vi "Report - PWP Stabilization Report.vi"(8 "error in":errorcluster, 11 "Fileid":string) -> (0 "error out":errorcluster)   [LabVIEW 2019]
uses:
  Controls/Report - State.ctl
  Controls/Report - Data Structure.ctl
  <vilib>/httpClient/ClientHandle.ctl
  Controls/FGV States.ctl
  Controls/eFGV States.ctl
  Controls/JSON - Fileid.ctl
  Controls/JSON - Report.ctl
  <vilib>/Utility/sysdir.llb/System Directory Type.ctl
  <vilib>/httpClient/POSTBuffer.vi
  <userlib>/_OpenG.lib/array/array.llb/Remove Duplicates from 1D Array (String)__ogtk.vi
  <userlib>/_OpenG.lib/array/array.llb/Delete Elements from 1D Array (String)__ogtk.vi
  <vilib>/Utility/config.llb/Read Key (String).vi
  <vilib>/httpClient/LabVIEWHTTPClient.lvlib
  <vilib>/Utility/config.llb/NI_LVConfig.lvlib
panel:
  in  "Plot":bool
  out "Current stage":T1
  in  "Back":bool
  in  "Forward":bool
  in  "Pages":u32
  out "Total":u32
  out "data":T2(array[cluster])
  in  "Cancel":bool
  in  "Generate":bool
  in  "Search":string
  in  "Listbox":i32(listbox)=-1 caption="Select File to Export"
  # "of"
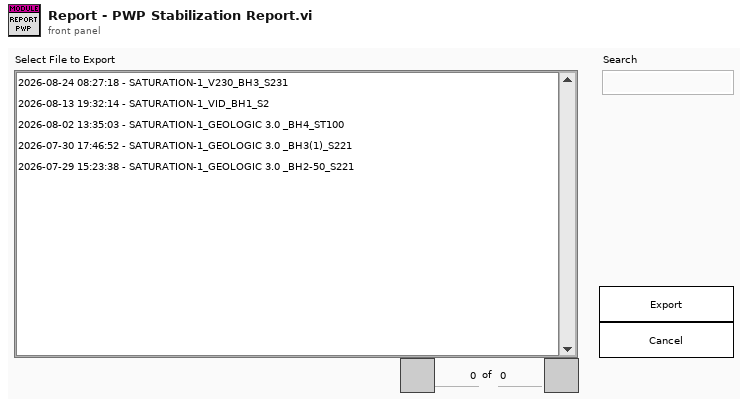
[diagram p1: front panel]
types:
  T1 = typedef "Report - State.ctl" = enum16{"Init", "Get File List", "Get Station Name", "Parse File List", "Idle", "Prepare to Generate", "Get Report", "Parse Report", "Get Data", "View T90", "Parse Data", "Convert to Excel", "Clean Up", "Close"}
  T2 = cluster{"id":string, "created_date":string, "testname":string, "jobno":string, "jobdesc":string, "sampleid":string, "date":string, "specimentno":string, "depth":string, "height":string, "diameter":string, "weight":string, "done":string}[]
  T3 = typedef "eFGV States.ctl" = enum16{"Init", "Read", "Write", "Exit"}
  T4 = typedef "FGV States.ctl" = enum16{"Read", "Write"}
  T5 = typedef "Report - Data Structure.ctl" = cluster{"API Ref":T6, "FileList":string[][], "Fileid":string, "testname":string[], "testtype":string[], "tdms":refnum<k34>, "TDMS Path":path, "tdms_path":string, "excel_path":string, "Excel Path":path, "List Name":string[], "Station Name":string[], "Plot":bool, "Tangent Point":string}
  T6 = typedef "LabVIEWHTTPClient.lvlib/ClientHandle.ctl" = refnum<k1>
  T7 = enum32{"Invalid", "Default", "Floating", "Floating/Auto-Hide", "Modal"}
  T8 = enum32{"Invalid", "Standard", "Closed", "Hidden", "Minimized", "Maximized"}
  T9 = typedef "JSON - Fileid.ctl" = cluster{"status":string, "data":cluster{"id":string, "created_date":string, "testname":string, "jobno":string, "jobdesc":string, "sampleid":string, "date":string, "specimentno":string, "depth":string, "height":string, "diameter":string, "weight":string, "done":string}[]}
  T10 = typedef "JSON - Report.ctl" = cluster{"status":string, "data":cluster{"testname":string, "testtype":string, "stage":string}[]}
  T11 = enum16{"open", "open or create", "create or replace", "create", "open (read-only)"}
  T12 = typedef "eventvkey.ctl" = enum16{"ASCII", "Enter", "Return", "Shift", "Ctrl", "Alt", "Cmd", "Opt", "Caps", "NumLock", "Clear", "Break", "Up", "Down", "Left", "Right", "Insert", "Delete", "Home", "End", "PageUp", "PageDown", "Escape", "Help", "Pause", "ScrollLock", "F1", "F2", "F3", "F4", "F5", "F6", "F7", "F8", "F9", "F10", "F11", "F12", "F13", "F14", "F15", "F16", "F17", "F18", "F19", "F20", "F21", "F22", "F23", "F24", "Play", "VolumeUp", "VolumeDown", "Mute", "Two Byte Char"}
  T13 = cluster{"testname":string, "testtype":string, "stage":string}[]
  T14 = typedef "System Directory Type.ctl" = i32
  T15 = typedef "NI_LVConfig.lvlib/Config Data RefNum.ctl" = refnum<k1>
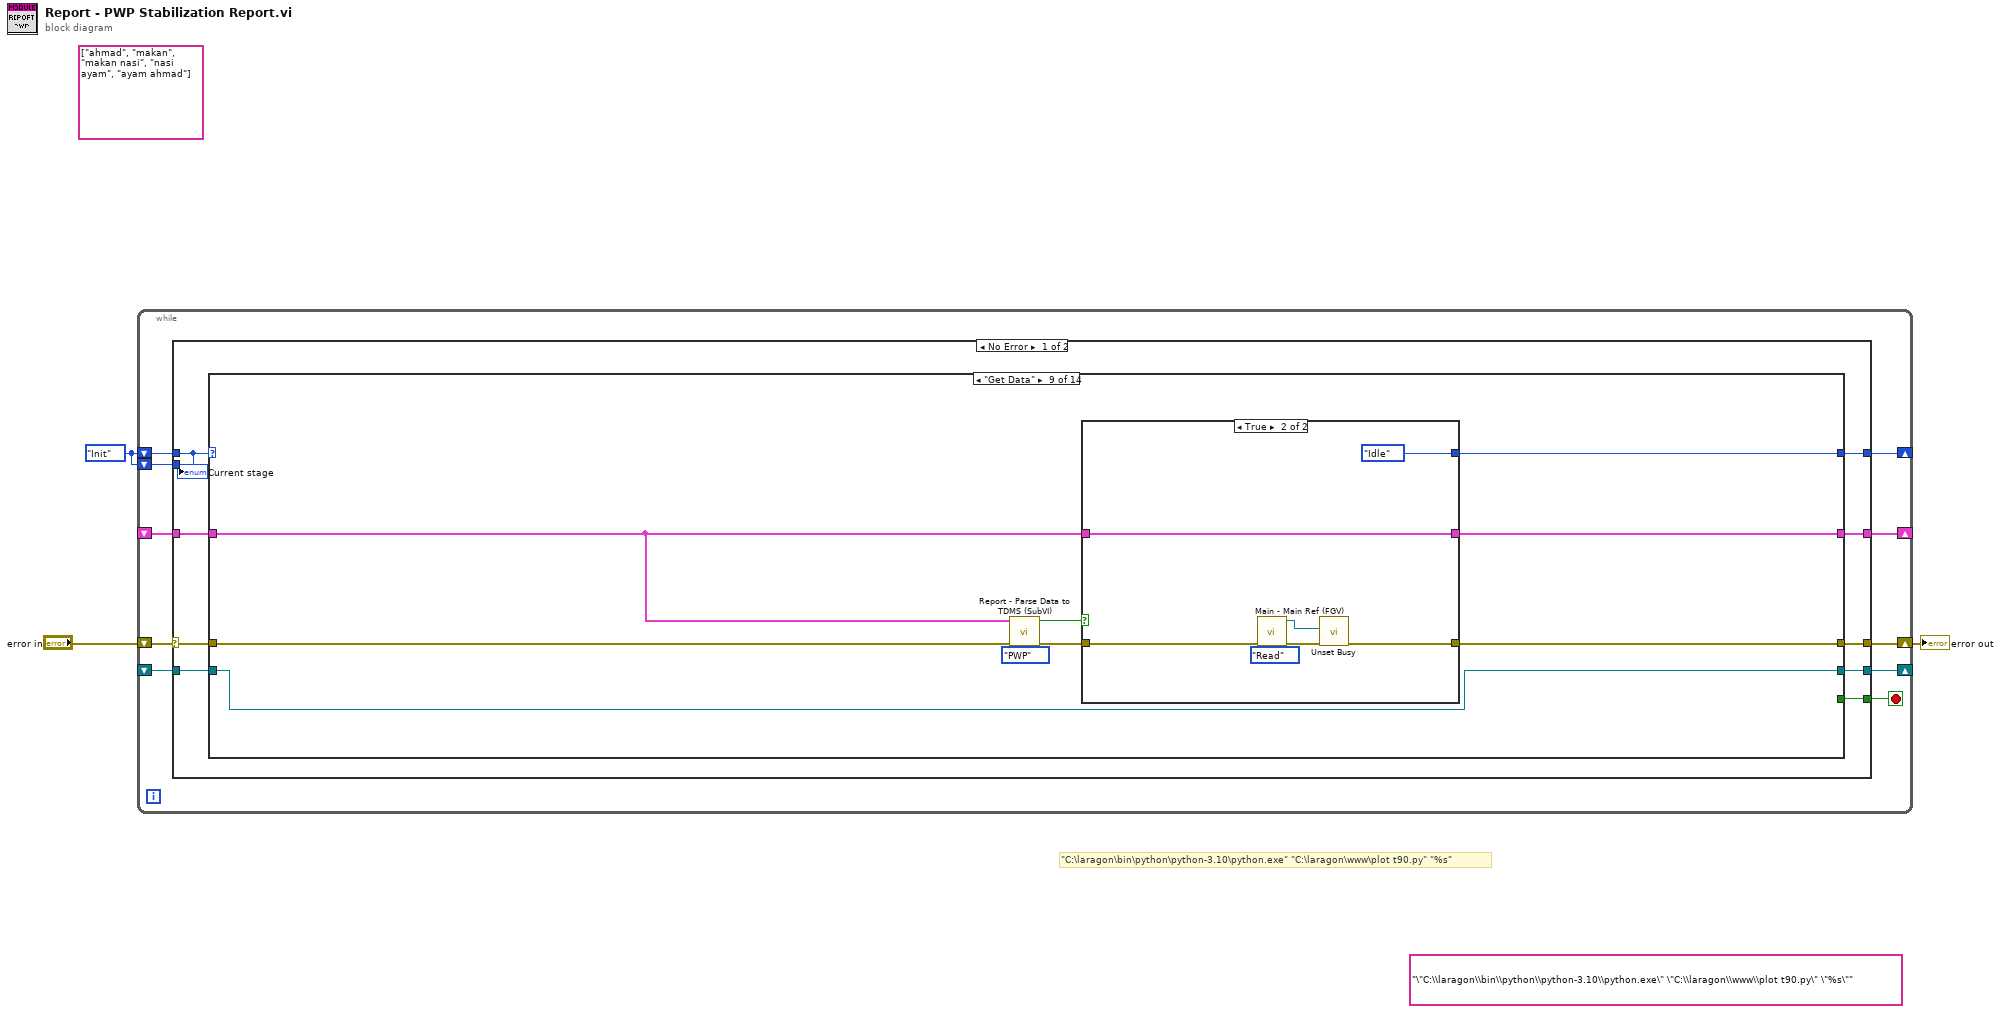
[diagram p0: block diagram]
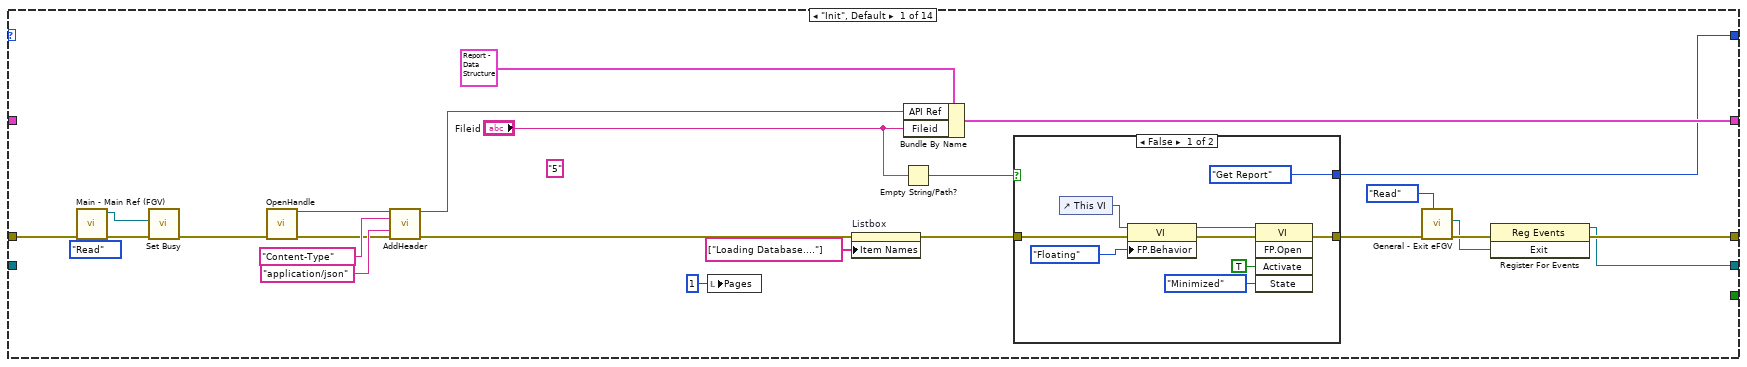
[diagram p2: hidden frame]
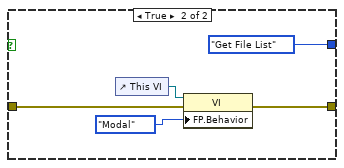
[diagram p3: hidden frame]
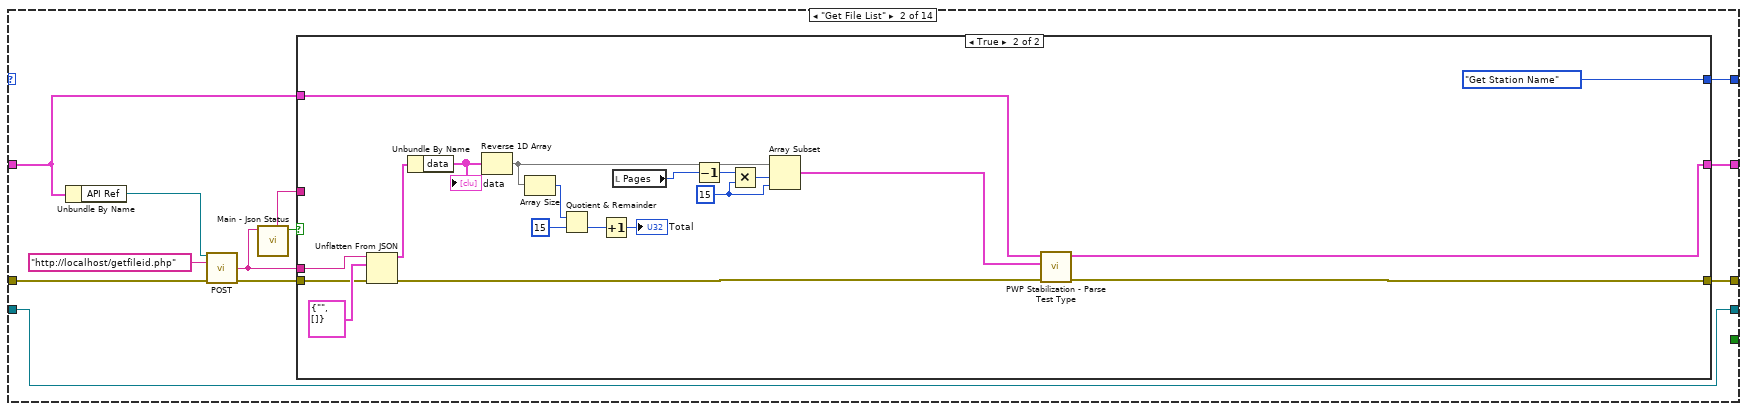
[diagram p4: hidden frame]
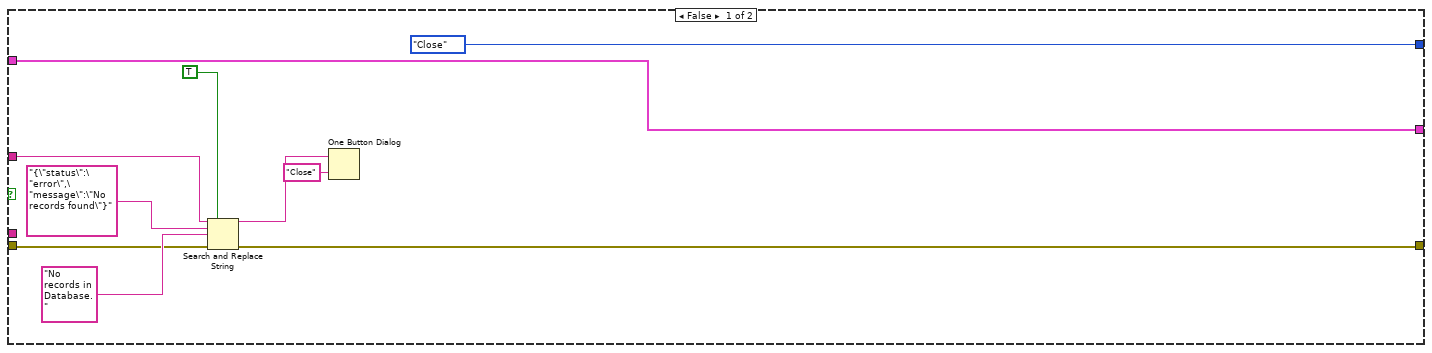
[diagram p5: hidden frame]
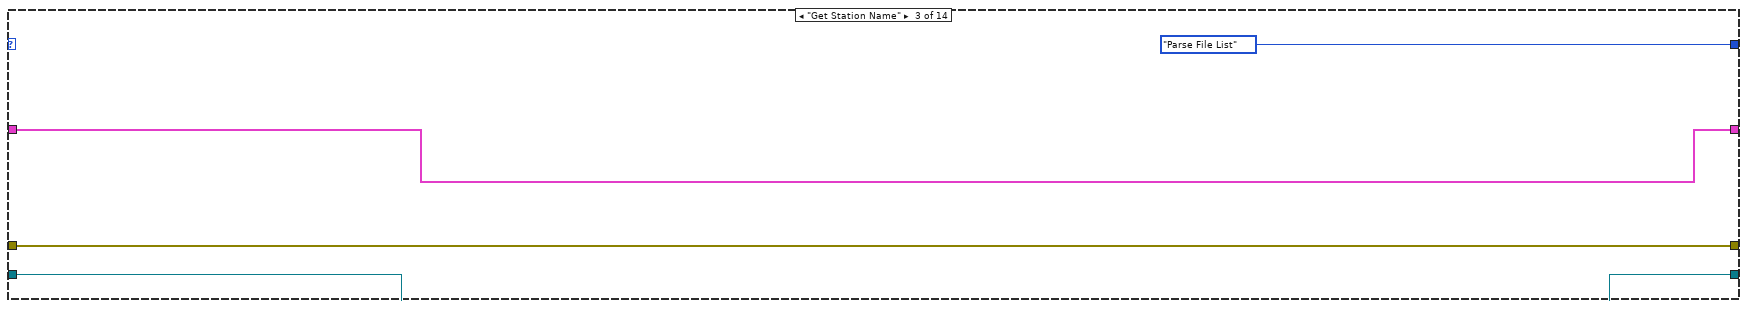
[diagram p6: hidden frame]
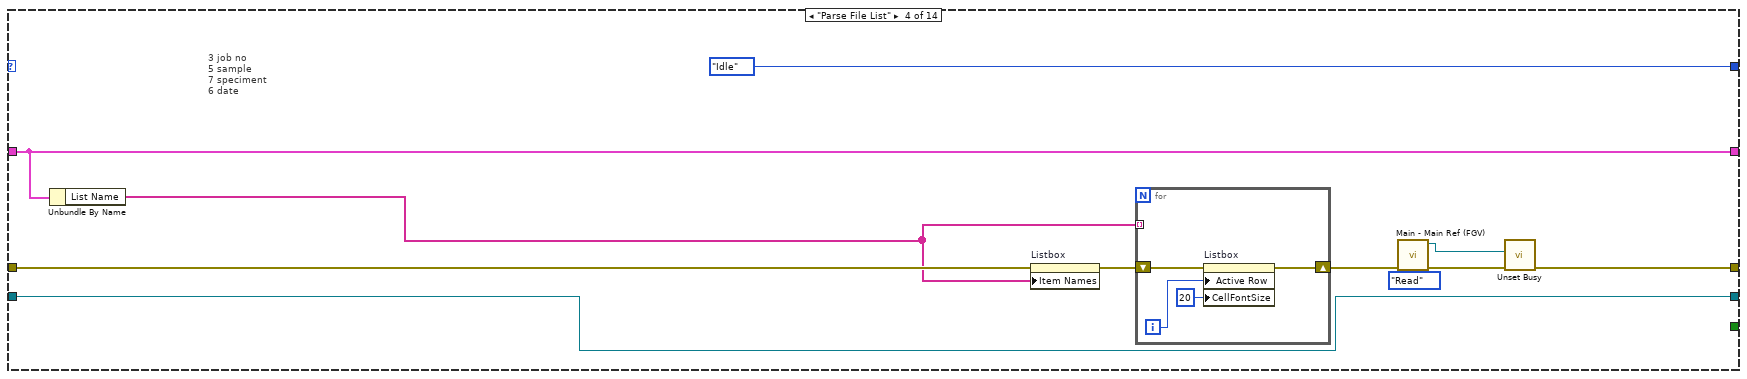
[diagram p7: hidden frame]
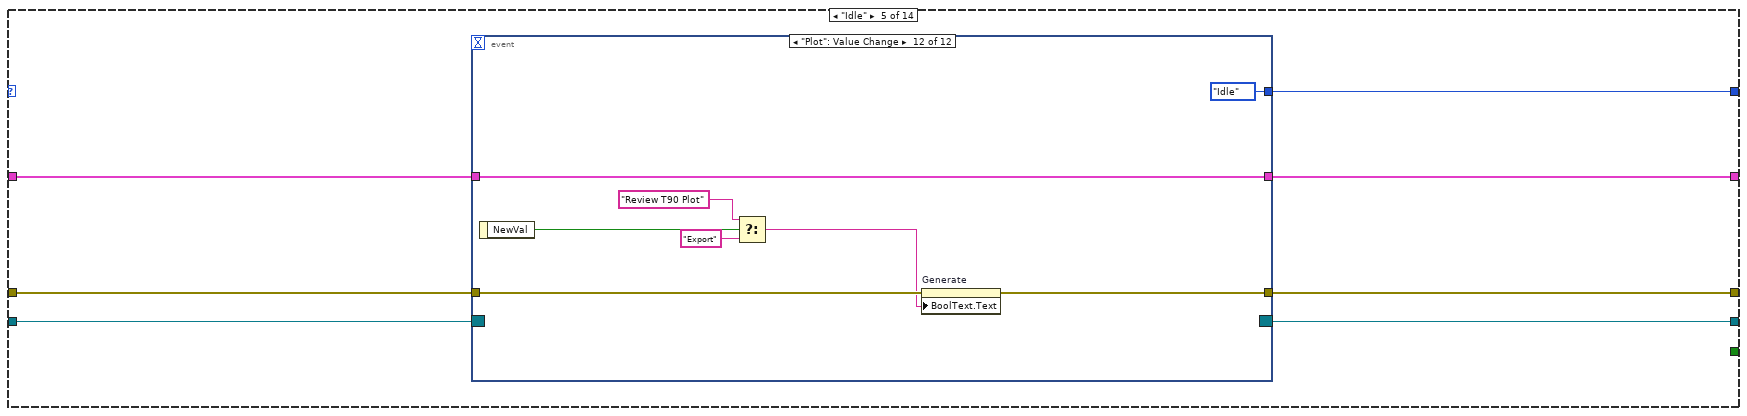
[diagram p8: hidden frame]
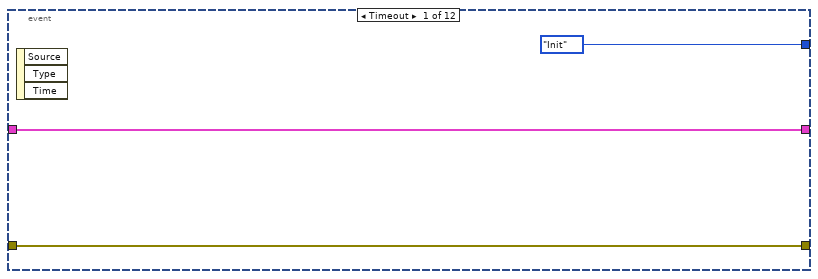
[diagram p9: hidden frame]
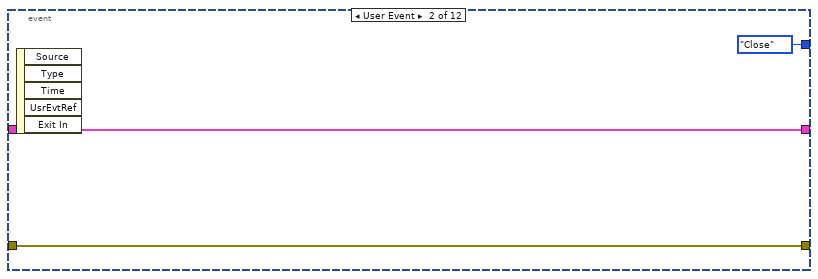
[diagram p10: hidden frame]
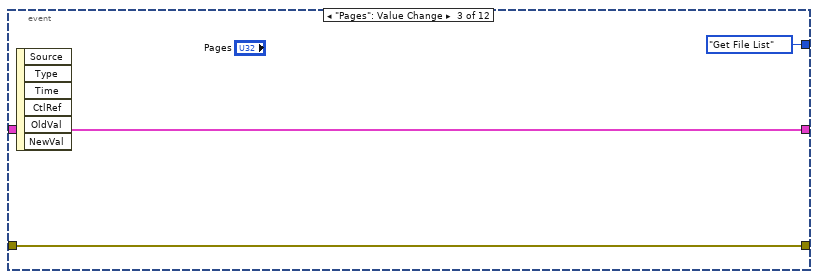
[diagram p11: hidden frame]
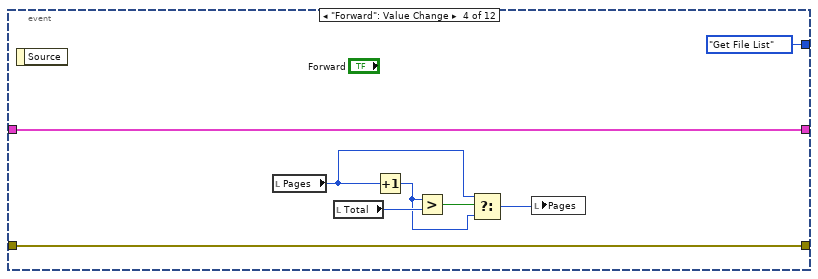
[diagram p12: hidden frame]
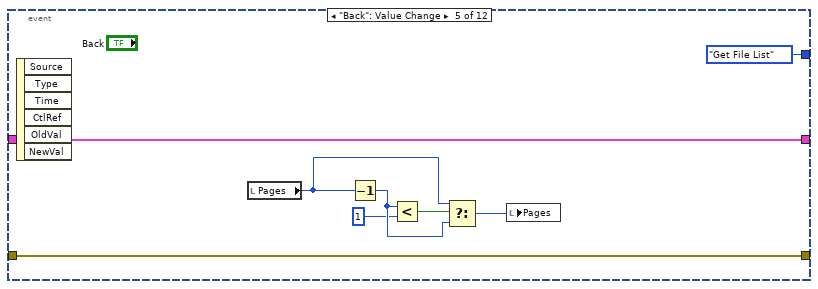
[diagram p13: hidden frame]
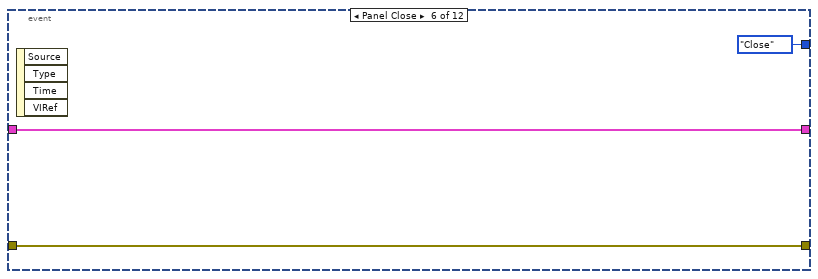
[diagram p14: hidden frame]
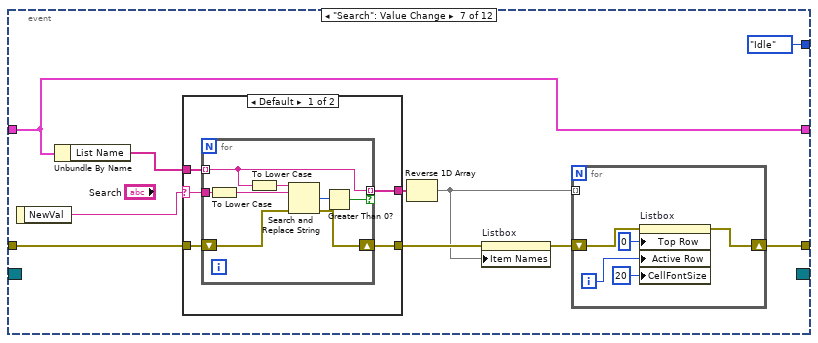
[diagram p15: hidden frame]
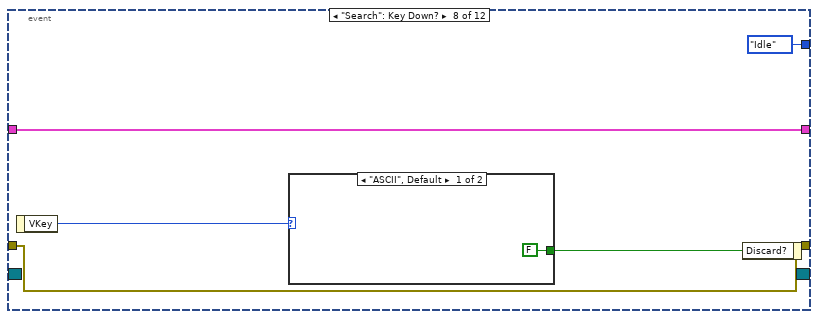
[diagram p17: hidden frame]
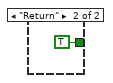
[diagram p18: hidden frame]
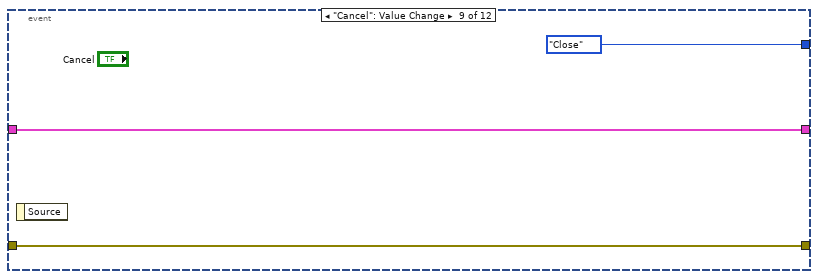
[diagram p19: hidden frame]
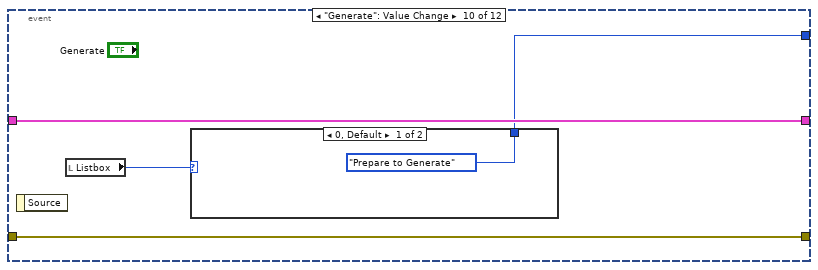
[diagram p20: hidden frame]
diagram:
  (unwired) "\"C:\\laragon\\bin\\python\\python-3.10\\python.exe\" \"C:\\laragon\\www\\plot t90.py\" \"%s\"" ("command line")
  w1 = Report_-_State."Init"
  (unwired) string[] ["ahmad", "makan", "makan nasi", "nasi ayam", "ayam ahmad"]
  # "\"C:\\laragon\\bin\\python\\python-3.10\\python.exe\" \"C:\\laragon\\www\\plot t90.py\" \"%s\""
  n1 = while {
    shift-right: [w10] -> w2
    shift-left: "error in" -> [w13]
    shift-right: [w11] -> _
    shift-left: w1 -> [w12]
    shift-right: [w9] -> _
    shift-left: _ -> [w8]
    shift-left: w1 -> [w6]
    shift-right: [w5] -> _
    shift-left: _ -> [w4]
    stop <- w7 stop-if-true
    n2 = case shown="No Error" w13 {
      selector: w13 -> [w20 w521]
      tunnel: w12 -> [w22 _]
      tunnel: [w21 Report_-_State."Close"] -> w11
      tunnel: [w19 w518] -> w10
      tunnel: [w18 w519] -> w9
      tunnel: w8 -> [w17 w519]
      tunnel: [w16 _] -> w7
      tunnel: w6 -> [_ w512]
      tunnel: [w15 w508] -> w5
      tunnel: w4 -> [w14 w508]
      frame No Error {
        n3 = case shown="\"Get Data\"" w22 {
          tunnel: [w40 w71 Report_-_State."Parse File List" Report_-_State."Idle" w127 Report_-_State."Get Report" w253 Report_-_State."Get Data" w318 Report_-_State."Parse Data" w358 w403 Report_-_State."Close" Report_-_State."Idle"] -> w21
          tunnel: w20 -> [w35 w72 w107 w117 w129 w236 w266 w304 w319 w346 w351 w399 w467 w504]
          tunnel: [w29 w69 w107 w111 w128 w250 w257 w301 w315 w345 w356 w407 w472 w496] -> w19
          tunnel: [w41 w66 w105 w115 w125 w241 w258 w300 w313 w341 w360 w406 w471 T5 {"API Ref"=refnum, "FileList"=[], "Fileid"="", "testname"=[], "testtype"=[], "tdms"=refnum, "TDMS Path"=path "", "tdms_path"="", "excel_path"="", "Excel Path"=path "", "List Name"=[], "Station Name"=[], "Plot"=FALSE, "Tangent Point"=""}] -> w18
          tunnel: w17 -> [_ w67 w105 w115 w126 w240 w260 w303 w312 w340 w363 w406 w471 w503]
          tunnel: [_ _ _ _ _ _ _ _ _ _ _ _ _ TRUE] -> w16
          tunnel: [w27 w62 w104 w108 w123 w233 w252 w296 w314 w347 w348 w387 w458 w495] -> w15
          tunnel: w14 -> [_ w62 w104 w108 w124 w233 w252 w296 w314 w347 w348 w387 w458 w495]
          frame "Init", Default {
            (unwired) "5"
            n4 = call "Main - Main Ref (FGV).vi"("Action"=FGV_States."Read", "error in"=w35) -> ("error out"=w36:errorcluster, "This VI out"=w34:refnum<vi>)  [unwired: 8 in]
            n5 = call <vilib>:"Set Busy.vi"("error in (no error)"=w36, "VI reference (current VI)"=w34) -> ("error out"=w38:errorcluster)  [unwired: 8 in, 1 out]
            n6 = call <vilib>:"OpenHandle.vi"("error in (no error)"=w38) -> ("client handle out"=w45:T6, "error out"=w44:errorcluster)  [unwired: 13 in]
            n7 = call <vilib>:"AddHeader.vi"("client handle"=w45, "header"="Content-Type", "value"="application/json", "error in (no error)"=w44) -> ("client handle out"=w42:T6, "error out"=w26:errorcluster)  [unwired: 10 in]
            n8 = local write "Pages"(u32 1 ("Pages")) -> ()
            n9 = property on="Listbox" class="LstBox (strict)"(error in=w26, "Item Names"=string[] ["Loading Database...."]) -> (error out=w25:errorcluster)  [unwired: 1 in, 1 out]
            n10 = Empty String/Path?(string/path="Fileid") -> (empty?=w39:bool)
            n11 = Bundle By Name(cluster=T5 {"API Ref"=refnum, "FileList"=[], "Fileid"="", "testname"=[], "testtype"=[], "tdms"=refnum, "TDMS Path"=path "", "tdms_path"="", "excel_path"="", "Excel Path"=path "", "List Name"=[], "Station Name"=[], "Plot"=FALSE, "Tangent Point"=""}, "API Ref"=w42, "Fileid"="Fileid") -> (w41:T5)
            n12 = case shown="False" w39 {
              tunnel: [Report_-_State."Get Report" ("f") Report_-_State."Get File List" ("f")] -> w40
              tunnel: w25 -> [w52 w58]
              tunnel: [w50 w57] -> w32
              frame False {
                n13 = control-ref of="This VI"() -> (w49:refnum<vi>)
                n14 = property class="VI"(reference=w49, error in=w52, "FP.Behavior"=T7."Floating" ("Front Panel Window:Behavior")) -> (reference out=w48:refnum<vi>, error out=w51:errorcluster)
                n15 = invoke class="VI" method="FP.Open"(reference=w48, error in=w51, "Activate"=TRUE ("Activate?"), "State"=T8."Minimized") -> (error out=w50:errorcluster)  [unwired: 1 in, 4 out]
              }
              frame True {
                n16 = control-ref of="This VI"() -> (w60:refnum<vi>)
                n17 = property class="VI"(reference=w60, error in=w58, "FP.Behavior"=T7."Modal" ("Front Panel Window:Behavior")) -> (error out=w57:errorcluster)  [unwired: 1 out]
              }
            }
            n18 = call "General - Exit eFGV.vi"("eFGV States"=eFGV_States."Read", "error in (no error)"=w32) -> ("error out"=w31:errorcluster, "Exit"=w28:refnum<user-event>)  [unwired: 7 in, 1 out]
            n19 = register-events(error in=w31, w28) -> (reference out=w27:refnum<event-registration>, error out=w29:errorcluster)  [unwired: 1 in]
          }
          frame "Get File List" {
            n20 = Unbundle By Name(w67) -> ("API Ref"=w68:T6)
            n21 = call-poly <vilib>:"POST.vi"("client handle"=w68, "url"="http://localhost/getfileid.php", "error in (no error)"=w72) -> ("body"=w65:string, "error out"=w70:errorcluster)  [unwired: 9 in, 2 out]
            n22 = call "Main - Json Status.vi"("json"=w65) -> ("Success?"=w64:bool, "message"=w63:string)  [unwired: 9 in]
            n23 = case shown="True" w64 {
              tunnel: [Report_-_State."Close" Report_-_State."Get Station Name"] -> w71
              tunnel: w70 -> [w74 w101]
              tunnel: [w75 w96] -> w69
              tunnel: w65 -> [_ w100]
              tunnel: w67 -> [w82 w86]
              tunnel: [w82 w97] -> w66
              tunnel: w63 -> [w77 _]
              frame False {
                n24 = Search and Replace String(replace all?=TRUE ("replace all? (F)"), input string=w77, search string="{\"status\":\"error\",\"message\":\"No records found\"}", replace string="No records in Database." ("replace string (\"\")"), error in=w74) -> (result string=w78:string, error out=w75:errorcluster)  [unwired: 3 in, 2 out]
                n25 = One Button Dialog(message=w78, button name ("OK")="Close") -> ()  [unwired: 1 out]
              }
              frame True {
                w91 = 15 ("length")
                n26 = Unflatten From JSON(JSON string=w100, type and defaults=T9 {"status"="", "data"=[]}, error in (no error)=w101) -> (value=w98:T9, error out=w88:errorcluster)  [unwired: 4 in]
                n27 = Unbundle By Name(w98) -> ("data"=w99:T2)
                "data" <- w99
                n28 = Reverse 1D Array(array=w99) -> (reversed array=w84:T2)
                n29 = Array Size(array=w84) -> (size(s)=w94:i32)
                n30 = Quotient & Remainder(x=w94, y=15) -> (floor(x/y)=w95:i32)  [unwired: 1 out]
                n31 = Increment(x=w95) -> (x+1=→"Total":i32)
                n32 = local read "Pages"() -> (w89:u32)
                n33 = Decrement(x=w89) -> (x-1=w90:u32)
                n34 = Multiply(x=w90, y=w91) -> (x*y=w92:u32)
                n35 = Array Subset(array=w84, index=w92, length=w91) -> (w85:T2)
                n36 = call "PWP Stabilization - Parse Test Type.vi"("error in (no error)"=w88, "Array"=w85, "Cluster in"=w86) -> ("error out"=w96:errorcluster, "Cluster out"=w97:T5)  [unwired: 6 in, 1 out]
              }
            }
          }
          frame "Get Station Name" {
          }
          frame "Parse File List" {
            # "3 job no\n5 sample\n7 speciment\n6 date"
            n37 = Unbundle By Name(w115) -> ("List Name"=w109:string[])
            n38 = property on="Listbox" class="LstBox (strict)"(error in=w117, "Item Names"=w109) -> (error out=w116:errorcluster)  [unwired: 1 in, 1 out]
            n39 = for {
              shift-right: [w120] -> w113
              shift-left: w116 -> [w121]
              tunnel: w109 -> [_] mode=indexing
              i -> [w119]
              n40 = property on="Listbox" class="LstBox (strict)"(error in=w121, "Active Row"=w119, "CellFontSize"=u32 20 ("Active Row:Cell Font:Size")) -> (error out=w120:errorcluster)  [unwired: 1 in, 1 out]
            }
            n41 = call "Main - Main Ref (FGV).vi"("Action"=FGV_States."Read", "error in"=w113) -> ("error out"=w112:errorcluster, "This VI out"=w110:refnum<vi>)  [unwired: 8 in]
            n42 = call <vilib>:"Unset Busy.vi"("error in (no error)"=w112, "VI reference (current VI)"=w110) -> ("error out"=w111:errorcluster)  [unwired: 9 in]
          }
          frame "Idle" {
            n43 = event shown="[11] \"Plot\": Value Change" {
              selector: w124 -> [_ _ _ _ _ _ _ _ _ _ _ _]
              dyn-events: [_ _ _ _ _ _ _ _ _ _ _ _] -> w123
              timeout: _ -> [_ _ _ _ _ _ _ _ _ _ _ _]
              tunnel: w129 -> [w132 w135 w136 w144 w154 w155 w163 w188 w196 w200 w217 w228]
              tunnel: [w132 w135 w136 w144 w154 w155 w162 w188 w196 w200 w214 w229] -> w128
              tunnel: [Report_-_State."Init" Report_-_State."Close" ("f") Report_-_State."Get File List" ("f") Report_-_State."Get File List" ("f") Report_-_State."Get File List" ("f") Report_-_State."Close" Report_-_State."Idle" Report_-_State."Idle" ("f") Report_-_State."Close" w198 w205 Report_-_State."Idle" ("f")] -> w127
              tunnel: w126 -> [w130 w134 w138 w145 w153 w156 w160 w192 w197 w201 w220 w231]
              tunnel: [w130 w134 w138 w145 w153 w156 w160 w192 w197 w201 w220 w231] -> w125
              event Timeout {
                n44 = event-data() -> ()  [unwired: 1 in, 3 out]
              }
              event User Event {
                n45 = event-data() -> ()  [unwired: 1 in, 5 out]
              }
              event "Pages": Value Change {
                n46 = event-data() -> ()  [unwired: 1 in, 6 out]
              }
              event "Forward": Value Change {
                n47 = event-data() -> ()  [unwired: 1 in, 1 out]
                n48 = local read "Pages"() -> (w141:u32)
                n49 = local read "Total"() -> (w143:u32)
                n50 = Increment(x=w141) -> (x+1=w140:u32)
                n51 = Greater?(x=w140, y=w143) -> (0:w142:bool)
                n52 = Select(t=w141, s=w142, f=w140) -> (s? t:f=w139:u32)
                n53 = local write "Pages"(w139) -> ()
              }
              event "Back": Value Change {
                n54 = event-data() -> ()  [unwired: 1 in, 6 out]
                n55 = local read "Pages"() -> (w150:u32)
                n56 = Decrement(x=w150) -> (x-1=w149:u32)
                n57 = Less?(x=w149, y=u32 1) -> (x < y?=w151:bool)
                n58 = Select(t=w150, s=w151, f=w149) -> (s? t:f=w148:u32)
                n59 = local write "Pages"(w148) -> ()
              }
              event Panel Close {
                n60 = event-data() -> ()  [unwired: 1 in, 4 out]
              }
              event "Search": Value Change {
                n61 = event-data() -> ("NewVal"=w161:string)  [unwired: 1 in]
                n62 = Unbundle By Name(w160) -> ("List Name"=w158:string[])
                n63 = case shown="Default" w161 {
                  selector: w161 -> [w173 _]
                  tunnel: w158 -> [w177 w187]
                  tunnel: w163 -> [w176 w186]
                  tunnel: [w175 w186] -> w166
                  tunnel: [w174 w187] -> w164
                  frame Default {
                    n64 = for {
                      tunnel: w173 -> [w185]
                      tunnel: [w182] -> w174 mode=indexing if=w183
                      tunnel: w177 -> [w182] mode=indexing
                      shift-right: [w180] -> w175
                      shift-left: w176 -> [w181]
                      n65 = To Lower Case(string=w185) -> (all lower case string=w179:string)
                      n66 = To Lower Case(string=w182) -> (all lower case string=w178:string)
                      n67 = Search and Replace String(input string=w178, search string=w179, error in=w181) -> (number of replacements=w184:i32, error out=w180:errorcluster)  [unwired: 5 in, 2 out]
                      n68 = Greater Than 0?(x=w184) -> (x > 0?=w183:bool)
                    }
                  }
                  frame "" {
                  }
                }
                n69 = Reverse 1D Array(array=w164) -> (reversed array=w159:string[])
                n70 = property on="Listbox" class="LstBox (strict)"(error in=w166, "Item Names"=w159) -> (error out=w165:errorcluster)  [unwired: 1 in, 1 out]
                n71 = for {
                  shift-right: [w170] -> w162
                  shift-left: w165 -> [w171]
                  tunnel: w159 -> [_] mode=indexing
                  i -> [w169]
                  n72 = property on="Listbox" class="LstBox (strict)"(error in=w171, "Top Row"=0, "Active Row"=w169, "CellFontSize"=u32 20 ("Active Row:Cell Font:Size")) -> (error out=w170:errorcluster)  [unwired: 1 in, 1 out]
                }
              }
              event "Search": Key Down? {
                n73 = event-data() -> ("VKey"=w190:T12)  [unwired: 1 in]
                n74 = case shown="\"ASCII\", Default" w190 {
                  tunnel: [FALSE TRUE] -> w189
                  frame "ASCII", Default {
                  }
                  frame "Return" {
                  }
                }
                n75 = event-data("Discard?"=w189) -> ()  [unwired: 1 in, 1 out]
              }
              event "Cancel": Value Change {
                n76 = event-data() -> ()  [unwired: 1 in, 1 out]
              }
              event "Generate": Value Change {
                n77 = event-data() -> ()  [unwired: 1 in, 1 out]
                n78 = local read "Listbox"() -> (w199:i32)
                n79 = case shown="0, Default" w199 {
                  tunnel: [Report_-_State."Prepare to Generate" Report_-_State."Idle"] -> w198
                  frame 0, Default {
                  }
                  frame -1 {
                    n80 = One Button Dialog(message="Please select a file") -> ()  [unwired: 1 in, 1 out]
                  }
                }
              }
              event "Listbox": Double Click {
                n81 = event-data() -> ("Row"=w215:i32)  [unwired: 1 in]
                n82 = property on="Listbox" class="LstBox (strict)"(error in=w217) -> (error out=w218:errorcluster, "Item Names"=w216:string[])  [unwired: 1 in, 1 out]
                n83 = Index Array(array=w216, index=w215) -> (element=w213:string)
                n84 = Format Into String(format string="Generate report %s?" ("message"), initial string="", error in=w218, w213) -> (resulting string=w210:string, error out=w214:errorcluster)
                n85 = Two Button Dialog(message=w210, 2:"Yes" ("T button name (\"OK\")")) -> (T button?=w206:bool)  [unwired: 1 in]
                n86 = local read "Listbox"() -> (w219:i32)
                n87 = case shown="0, Default" w219 {
                  tunnel: [Report_-_State."Prepare to Generate" Report_-_State."Idle"] -> w208
                  frame 0, Default {
                  }
                  frame -1 {
                    n88 = One Button Dialog(message="Please select a file") -> ()  [unwired: 1 in, 1 out]
                  }
                }
                n89 = Select(t=w208, s=w206, f=Report_-_State."Idle") -> (s? t:f=w205:T1)
              }
              event "Plot": Value Change {
                n90 = event-data() -> ("NewVal"=w226:bool)  [unwired: 1 in]
                n91 = Select(t="Review T90 Plot" ("Boolean Text.Text"), s=w226, f="Export") -> (s? t:f=w224:string)
                n92 = property on="Generate" class="Bool"(error in=w228, "BoolText.Text"=w224) -> (error out=w229:errorcluster)  [unwired: 1 in, 1 out]
              }
            }
          }
          frame "Prepare to Generate" {
            n93 = call "Main - Main Ref (FGV).vi"("Action"=FGV_States."Read", "error in"=w236) -> ("error out"=w237:errorcluster, "This VI out"=w235:refnum<vi>)  [unwired: 8 in]
            n94 = call <vilib>:"Set Busy.vi"("error in (no error)"=w237, "VI reference (current VI)"=w235) -> ("error out"=w239:errorcluster)  [unwired: 8 in, 1 out]
            n95 = property on="Listbox" class="LstBox (strict)"(error in=w239) -> (error out=w250:errorcluster, "Item Names"=w248:string[])  [unwired: 1 in, 1 out]
            n96 = Unbundle By Name(w240) -> ("FileList"=w247:string[][], "List Name"=w234:string[])
            n97 = Index Array(array=w247, index (col)=0 ("disabled index (col)")) -> (element=w244:string[])  [unwired: 1 in]
            n98 = Index Array(array=w248, index="Listbox") -> (element=w245:string)
            n99 = Search 1D Array(1D array=w234, element=w245) -> (index of element=w243:i32)  [unwired: 1 in]
            n100 = Index Array(array=w244, index=w243) -> (element=w242:string)
            n101 = Bundle By Name(cluster=w240, "Plot"="Plot", "Fileid"=w242) -> (w241:T5)
          }
          frame "Get Report" {
            n102 = Unbundle By Name(w260) -> ("API Ref"=w259:T6, "Fileid"=w265:string)
            n103 = Bundle By Name(cluster=cluster{"fileid":string} {"fileid"=""}, "fileid"=w265) -> (w267:cluster{"fileid":string})
            n104 = Flatten To JSON(anything=w267, error in (no error)=w266) -> (JSON string=w262:string, 11:w263:errorcluster)  [unwired: 1 in]
            n105 = call-poly <vilib>:"POST.vi"("client handle"=w259, "url"="http://localhost/report.php", "buffer"=w262, "error in (no error)"=w263) -> ("body"=w256:string, "error out"=w261:errorcluster)  [unwired: 8 in, 2 out]
            n106 = call "Main - Json Status.vi"("json"=w256) -> ("Success?"=w255:bool, "message"=w254:string)  [unwired: 9 in]
            n107 = case shown="True" w255 {
              tunnel: w261 -> [w270 w286]
              tunnel: w260 -> [w273 w283]
              tunnel: [w273 w280] -> w258
              tunnel: [w269 w279] -> w257
              tunnel: w256 -> [_ w278]
              tunnel: w254 -> [w272 _]
              tunnel: [Report_-_State."Close" Report_-_State."Parse Report"] -> w253
              frame False {
                n108 = One Button Dialog(message=w272) -> ()  [unwired: 1 in, 1 out]
                n109 = call <vilib>:"Clear Errors.vi"("error in (no error)"=w270) -> ("error out"=w269:errorcluster)  [unwired: 5 in, 1 out]
              }
              frame True {
                n110 = Unflatten From JSON(JSON string=w278, type and defaults=T10 {"status"="", "data"=[]}, error in (no error)=w286) -> (value=w285:T10, error out=w279:errorcluster)  [unwired: 4 in]
                n111 = Unbundle By Name(w285) -> ("data"=w276:T13)
                n112 = for {
                  tunnel: w276 -> [w295] mode=indexing
                  tunnel: [w294] -> w275 mode=indexing
                  tunnel: [w291] -> w274 mode=indexing
                  n113 = Unbundle By Name(w295) -> ("testtype"=w294:string, "testname"=w293:string, "stage"=w290:string)
                  n114 = Match Pattern(string=w290, regular expression="Test Stage ") -> (after substring=w288:string)  [unwired: 1 in, 3 out]
                  n115 = Concatenate Strings(w293, " | " ("string"), w288) -> (w291:string)
                }
                n116 = call-poly <userlib>:"Remove Duplicates from 1D Array__ogtk.vi"("Input Array"=w274) -> ("Output Array"=w281:string[], "indices of removed elements"=w284:i32[])
                n117 = call-poly <userlib>:"Delete Elements from Array__ogtk.vi"("indices"=w284, "array"=w275) -> ("array w/ subset deleted"=w282:string[])  [unwired: 8 in, 1 out]
                n118 = Bundle By Name(cluster=w283, "testtype"=w282, "testname"=w281) -> (w280:T5)
              }
            }
          }
          frame "Parse Report" {
            n119 = Format Date/Time String(time format string (%c)="%H%M%S") -> (date/time string=w307:string)  [unwired: 2 in]
            n120 = Concatenate Strings("convert-" ("string"), w307, ".tdms" ("string")) -> (w305:string)
            n121 = Temporary Directory() -> (w297:path)
            n122 = Build Path(base path=w297, name or relative path=w305) -> (appended path=w298:path)
            n123 = TDMS Open(8:w304, 10:T11."create" ("operation (0:open)"), 11:w298) -> (0:w301:errorcluster, 3:w302:refnum<k34>)  [unwired: 4 in]
            n124 = Bundle By Name(cluster=w303, "TDMS Path"=w298, "tdms"=w302) -> (w300:T5)
          }
          frame "Get Data" {
            n125 = call "Report - Parse Data to TDMS (SubVI).vi"("error in (no error)"=w319, "Enum"=enum16{"Report", "PWP"}."PWP", "Cluster"=w312) -> ("error out"=w316:errorcluster, "Cancel?"=w317:bool)  [unwired: 7 in]
            n126 = case shown="True" w317 {
              tunnel: [w324 Report_-_State."Idle"] -> w318
              tunnel: w316 -> [w322 w335]
              tunnel: [w323 w334] -> w315
              tunnel: [w321 w333] -> w313
              tunnel: w312 -> [w321 w333]
              frame False {
                n127 = Unbundle By Name(w321) -> ("Plot"=w320:bool)
                n128 = case shown="True" w320 {
                  tunnel: [Report_-_State."Parse Data" Report_-_State."View T90"] -> w324
                  tunnel: [w326 w328] -> w323
                  tunnel: w322 -> [w326 w327]
                  frame False {
                  }
                  frame True {
                    n129 = call "Main - Main Ref (FGV).vi"("Action"=FGV_States."Read", "error in"=w327) -> ("error out"=w330:errorcluster, "This VI out"=w329:refnum<vi>)  [unwired: 8 in]
                    n130 = call <vilib>:"Unset Busy.vi"("error in (no error)"=w330, "VI reference (current VI)"=w329) -> ("error out"=w328:errorcluster)  [unwired: 9 in]
                  }
                }
              }
              frame True {
                n131 = call "Main - Main Ref (FGV).vi"("Action"=FGV_States."Read", "error in"=w335) -> ("error out"=w337:errorcluster, "This VI out"=w336:refnum<vi>)  [unwired: 8 in]
                n132 = call <vilib>:"Unset Busy.vi"("error in (no error)"=w337, "VI reference (current VI)"=w336) -> ("error out"=w334:errorcluster)  [unwired: 9 in]
              }
            }
          }
          frame "View T90" {
            n133 = Unbundle By Name(w340) -> ("Fileid"=w343:string)
            n134 = call "Run Test - T90 Plot (SubVI).vi"("error in (no error)"=w346, "fileid"=w343) -> ("error out"=w345:errorcluster, "Tengent Point"=w342:string)  [unwired: 8 in]
            n135 = Bundle By Name(cluster=w340, "Tangent Point"=w342) -> (w341:T5)
          }
          frame "Parse Data" {
            w367 = T14 1 items=["User Home"=0, "User Desktop"=1, "User Documents"=2, "User Application Data"=3, "User Preferences"=4, "User Temporary"=5, "Public Documents"=6, "Public Application Data"=7, "Public Preferences"=8, "Public Cache"=13, "System Core Libraries"=9, "System Installed Libraries"=10, "Application Files"=11, "Boot Volume Root"=12] ("system directory type")
            n136 = Unbundle By Name(w363) -> ("TDMS Path"=w364:path)
            n137 = call "Main - Main Ref (FGV).vi"("Action"=FGV_States."Read", "error in"=w351) -> ("error out"=w352:errorcluster, "This VI out"=w349:refnum<vi>)  [unwired: 8 in]
            n138 = call <vilib>:"Unset Busy.vi"("error in (no error)"=w352, "VI reference (current VI)"=w349) -> ("error out"=w350:errorcluster)  [unwired: 9 in]
            n139 = call <vilib>:"Get System Directory.vi"("system directory type"=w367) -> ("system directory"=w359:path)  [unwired: 10 in]
            n140 = call "File Dialog"("start path"=w359, "error in"=w350, "pattern (all files)"="*.xlsx", "pattern label"=".xlsx") -> ("selected path"=w354:path, "cancelled"=w357:bool, "error out"=w355:errorcluster)  [unwired: 8 in, 1 out]
            n141 = Path To String(path=w364) -> (string=w362:string)
            n142 = Path To String(path=w354) -> (string=w361:string)
            n143 = case shown="False" w357 {
              tunnel: w363 -> [w374 _]
              tunnel: w362 -> [w373 _]
              tunnel: w361 -> [w372 _]
              tunnel: [w371 T5 {"API Ref"=refnum, "FileList"=[], "Fileid"="", "testname"=[], "testtype"=[], "tdms"=refnum, "TDMS Path"=path "", "tdms_path"="", "excel_path"="", "Excel Path"=path "", "List Name"=[], "Station Name"=[], "Plot"=FALSE, "Tangent Point"=""}] -> w360
              tunnel: [Report_-_State."Convert to Excel" Report_-_State."Close"] -> w358
              tunnel: [w369 w375] -> w356
              tunnel: w355 -> [w369 w376]
              tunnel: w354 -> [w368 _]
              frame False {
                n144 = Bundle By Name(cluster=w374, "tdms_path"=w373, "excel_path"=w372, "Excel Path"=w368) -> (w371:T5)
              }
              frame True {
                n145 = call <vilib>:"Clear Errors.vi"("error in (no error)"=w376) -> ("error out"=w375:errorcluster)  [unwired: 5 in, 1 out]
              }
            }
          }
          frame "Convert to Excel" {
            n146 = Unbundle By Name(w406) -> ("Plot"=w380:bool, "TDMS Path"=w392:path, "API Ref"=w412:T6, "tdms_path"=w417:string, "excel_path"=w381:string, "Tangent Point"=w379:string)
            n147 = Path To String(path=w392) -> (string=w391:string)
            n148 = call "Main - Main Ref (FGV).vi"("Action"=FGV_States."Read", "error in"=w399) -> ("error out"=w400:errorcluster, "This VI out"=w397:refnum<vi>)  [unwired: 8 in]
            n149 = Concatenate Strings(w391, "_index" ("string")) -> (w389:string)
            n150 = call <vilib>:"Set Busy.vi"("error in (no error)"=w400, "VI reference (current VI)"=w397) -> ("error out"=w398:errorcluster)  [unwired: 8 in, 1 out]
            n151 = Bundle By Name(cluster=cluster{"tdms_path":string, "excel_path":string} {"tdms_path"="", "excel_path"=""}, "tdms_path"=w417, "excel_path"=w381) -> (w422:cluster{"tdms_path":string, "excel_path":string})
            n152 = String To Path(string=w389) -> (path=w388:path)
            n153 = Flatten To JSON(anything=w422, error in (no error)=w398) -> (JSON string=w419:string, 11:w416:errorcluster)  [unwired: 1 in]
            n154 = Search and Replace String(replace all?=TRUE ("replace all? (F)"), input string=w419, search string="\\\\", replace string="/" ("replace string (\"\")"), error in=w416) -> (result string=w413:string, error out=w415:errorcluster)  [unwired: 3 in, 2 out]
            n155 = call-poly <vilib>:"POST.vi"("client handle"=w412, "url"="http://localhost/convert.php", "buffer"=w413, "error in (no error)"=w415) -> ("body"=w385:string, "error out"=w408:errorcluster)  [unwired: 8 in, 2 out]
            n156 = Search and Replace String(input string=w385, search string="\"status\":\"success\"", error in=w408) -> (number of replacements=w410:i32, error out=w383:errorcluster)  [unwired: 5 in, 2 out]
            n157 = Unbundle By Name(w383) -> ("source"=w382:string)
            n158 = Greater Than 0?(x=w410) -> (x > 0?=w409:bool)
            n159 = call "Main - Main Ref (FGV).vi"("Action"=FGV_States."Read", "error in"=w383) -> ("error out"=w395:errorcluster, "This VI out"=w393:refnum<vi>)  [unwired: 8 in]
            n160 = call <vilib>:"Unset Busy.vi"("error in (no error)"=w395, "VI reference (current VI)"=w393) -> ("error out"=w394:errorcluster)  [unwired: 9 in]
            n161 = Concatenate Strings(w382, ", Body: " ("string"), w385) -> (w384:string)
            n162 = case shown="False" w409 {
              tunnel: w392 -> [_ w444]
              tunnel: w394 -> [w428 w443]
              tunnel: [w429 w435] -> w407
              tunnel: [FALSE ("T button?") w439] -> w405
              tunnel: w388 -> [_ w437]
              tunnel: w384 -> [w424 _]
              tunnel: w381 -> [_ w434]
              tunnel: w380 -> [_ w433]
              tunnel: w379 -> [_ w432]
              frame False {
                n163 = Format Into String(format string="There is an error to generate your report.\n\n%s" ("message"), initial string="", error in=w428, w424) -> (resulting string=w426:string, error out=w429:errorcluster)
                n164 = One Button Dialog(message=w426, button name ("OK")="Close") -> ()  [unwired: 1 out]
              }
              frame True {
                n165 = Delete(path (use dialog)=w444, error in=w443) -> (error out=w438:errorcluster)  [unwired: 3 in, 2 out]
                n166 = Delete(path (use dialog)=w437, error in=w438) -> (error out=w436:errorcluster)  [unwired: 3 in, 2 out]
                n167 = case shown="True" w433 {
                  tunnel: w436 -> [w445 w451]
                  tunnel: [w445 w452] -> w435
                  tunnel: w434 -> [_ w449]
                  tunnel: w432 -> [_ w446]
                  frame False {
                  }
                  frame True {
                    (unwired) " \"3,4\"" ("string")
                    w448 = "\"" ("string")
                    n168 = Concatenate Strings("\"C:\\laragon\\bin\\python\\python-3.10\\python.exe\" \"C:\\laragon\\www\\plot t90 v2.py\" " ("command line"), w448, w449, w448, w446) -> (w447:string)
                    n169 = call <vilib>:"System Exec.vi"("run minimized? (F)"=TRUE, "wait until completion? (T)"=TRUE, "error in (no error)"=w451, "command line"=w447) -> ("error out"=w452:errorcluster)  [unwired: 4 in, 3 out]
                  }
                }
                n170 = Two Button Dialog(message="Your report has been generated.\nLoad file now?", 1:"No" ("F button name (\"Cancel\")"), 2:"Yes" ("T button name (\"OK\")")) -> (T button?=w439:bool)
              }
            }
            n171 = Select(t=Report_-_State."Clean Up", s=w405, f=Report_-_State."Close") -> (s? t:f=w403:T1)
          }
          frame "Clean Up" {
            (unwired) path "C:/Program Files/Microsoft Office/root/Office16/EXCEL.EXE"
            # "- Consolidation report.xlsx"
            n172 = Unbundle By Name(w471) -> ("Plot"=w455:bool, "Excel Path"=w457:path)
            n173 = case shown="False" w455 {
              tunnel: w457 -> [w474 w482]
              tunnel: [w474 w475] -> w456
              frame False {
              }
              frame True {
                n174 = Strip Path(path=w482) -> (stripped path=w477:path, name=w481:string)
                n175 = Match Pattern(string=w481, regular expression=".xlsx") -> (before substring=w479:string)  [unwired: 1 in, 3 out]
                n176 = Concatenate Strings(w479, " - Consolidation report.xlsx" ("regular expression")) -> (w476:string)
                n177 = Build Path(base path=w477, name or relative path=w476) -> (appended path=w475:path)
              }
            }
            n178 = call <vilib>:"Application Directory.vi"() -> ("Application Directory"=w470:path)
            n179 = Build Path(base path=w470, name or relative path="Data\\.env") -> (appended path=w468:path)
            n180 = call <vilib>:"Open Config Data.vi"("error in (no error)"=w467, "configuration file path"=w468) -> ("error out"=w466:errorcluster, "refnum"=w465:T15)  [unwired: 7 in, 1 out]
            n181 = call-poly <vilib>:"Read Key.vi"("section"="Excel" ("key"), "error in (no error)"=w466, "key"="Path" ("default value"), "refnum"=w465) -> ("error out"=w464:errorcluster, "value"=w459:string, "refnum out"=w463:T15)  [unwired: 4 in, 1 out]
            n182 = call <vilib>:"Close Config Data.vi"("error in (no error)"=w464, "refnum"=w463) -> ("error out"=w462:errorcluster)  [unwired: 8 in, 1 out]
            n183 = case shown="Default" w459 {
              tunnel: [w486 w493] -> w472
              tunnel: w456 -> [w485 _]
              tunnel: w459 -> [w484 _]
              tunnel: w462 -> [w483 w493]
              frame Default {
                n184 = Format Into String(format string="\"%s\" \"%s\"" ("command line"), error in=w483, w484, w485) -> (resulting string=w488:string, error out=w487:errorcluster)  [unwired: 1 in]
                n185 = call <vilib>:"System Exec.vi"("run minimized? (F)"=TRUE, "wait until completion? (T)"=FALSE, "error in (no error)"=w487, "command line"=w488) -> ("error out"=w486:errorcluster)  [unwired: 4 in, 3 out]
              }
              frame "" {
                n186 = One Button Dialog(message="Please set excel path in .env file") -> ()  [unwired: 1 in, 1 out]
              }
            }
          }
          frame "Close" {
            n187 = Unbundle By Name(w503) -> ("API Ref"=w502:T6)
            n188 = call <vilib>:"CloseHandle.vi"("client handle"=w502, "error in (no error)"=w504) -> ("error out"=w498:errorcluster)  [unwired: 13 in]
            n189 = call "Main - Main Ref (FGV).vi"("Action"=FGV_States."Read", "error in"=w498) -> ("error out"=w500:errorcluster, "This VI out"=w499:refnum<vi>)  [unwired: 8 in]
            n190 = call <vilib>:"Unset Busy.vi"("error in (no error)"=w500, "VI reference (current VI)"=w499) -> ("error out"=w497:errorcluster)  [unwired: 9 in]
            n191 = control-ref of="This VI"() -> (w494:refnum<vi>)
            n192 = invoke class="VI" method="FP.Close"(reference=w494, error in=w497) -> (error out=w496:errorcluster)  [unwired: 1 in, 2 out]
          }
        }
        "Current stage" <- w22
      }
      frame Error {
        n193 = Unbundle By Name(w521) -> ("source"=w515:string)
        n194 = call <vilib>:"Clear Errors.vi"("error in (no error)"=w521) -> ("error out"=w514:errorcluster)  [unwired: 5 in, 1 out]
        n195 = Format Into String(error in=w514, w512) -> (resulting string=w509:string, error out=w513:errorcluster)  [unwired: 2 in]
        n196 = Concatenate Strings(w515, "\n" ("string"), w509) -> (w511:string)
        n197 = call "Main - Main Ref (FGV).vi"("Action"=FGV_States."Read", "error in"=w513) -> ("error out"=w523:errorcluster, "This VI out"=w522:refnum<vi>)  [unwired: 8 in]
        n198 = call <vilib>:"Unset Busy.vi"("error in (no error)"=w523, "VI reference (current VI)"=w522) -> ("error out"=w520:errorcluster)  [unwired: 9 in]
        n199 = flat-sequence {
          tunnel: w511 -> [w528]
          tunnel: [w527] -> w517
          tunnel: w520 -> [w527]
          frame #0 {
            n200 = One Button Dialog(message=w528) -> ()  [unwired: 1 in, 1 out]
          }
        }
        n201 = Unbundle By Name(w519) -> ("API Ref"=w516:T6)
        n202 = call <vilib>:"CloseHandle.vi"("client handle"=w516, "error in (no error)"=w517) -> ("error out"=w518:errorcluster)  [unwired: 13 in]
        n203 = Wait (ms)(milliseconds to wait=u32 1000) -> ()  [unwired: 1 out]
      }
    }
  }
  "error out" <- w2
